vi "TCatAdsNetLibraryTester.vi"() -> ()   [LabVIEW 2016, in "TCatAdsNet.lvlib"]
uses:
  TCatAdsNet.lvlib
  AdsNET.lvclass
panel:
  out "Catalog Elapsed Time (ms)":u32
  out "Elapsed Time (ms)":u32
  out "Values (SGL)":sgl[](array[numeric])
  out "error out":errorcluster
  out "Value":string
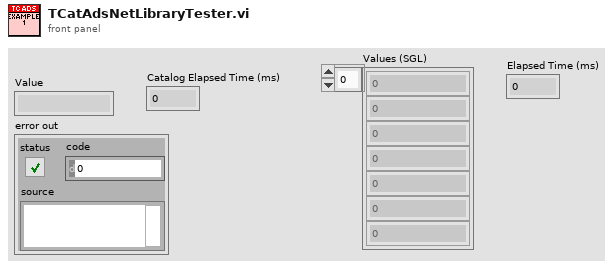
[diagram p1: front panel]
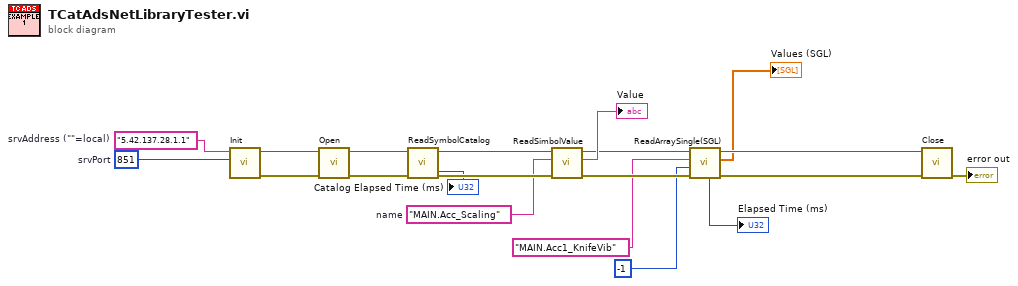
[diagram p0: block diagram]
diagram:
  w12 = "MAIN.Acc_Scaling"  # name
  w13 = 851  # srvPort
  w14 = "5.42.137.28.1.1"  # srvAddress (""=local)
  n1 = call "Init.vi"("srvPort"=w13, "srvAddress (\"\"=local)"=w14) -> ("error out"=w20:errorcluster, "TCatAdsNet"=w19:refnum<class "AdsNET.lvclass">)  [unwired: 8 in]
  n2 = call "Open.vi"("error in (no error)"=w20, "TCatAdsNet in"=w19) -> ("error out"=w18:errorcluster, "TCatAdsNet out"=w17:refnum<class "AdsNET.lvclass">)  [unwired: 8 in]
  n3 = call "ReadSymbolCatalog.vi"("error in (no error)"=w18, "AdsNET in"=w17) -> ("error out"=w15:errorcluster, "AdsNET out"=w16:refnum<class "AdsNET.lvclass">, "Elapsed Time (ms)"=→"Catalog Elapsed Time (ms)":u32)  [unwired: 7 in]
  n4 = call "ReadSimbolValue.vi"("error in (no error)"=w15, "name"=w12, "TCatAdsNet in"=w16) -> ("error out"=w9:errorcluster, "Value"=→"Value":string, "TCatAdsNet out"=w7:refnum<class "AdsNET.lvclass">)  [unwired: 4 in, 2 out]
  n5 = call "ReadArraySingle(SGL).vi"("error in (no error)"=w9, "Elements (-1 = auto)"=-1, "variableName"="MAIN.Acc1_KnifeVib", "TCatAdsNet in"=w7) -> ("error out"=w8:errorcluster, "Values (SGL)"=→"Values (SGL)":sgl[], "TCatAdsNet out"=w6:refnum<class "AdsNET.lvclass">, "Elapsed Time (ms)"=→"Elapsed Time (ms)":u32)  [unwired: 3 in, 1 out]
  n6 = call "Close.vi"("error in (no error)"=w8, "TCatAdsNet in"=w6) -> ("error out"=→"error out":errorcluster)  [unwired: 9 in]
